vi "Th 1tache.vi"(3 "Indice tache":i8) -> (0 "données Th":string[](array[string]))   [LabVIEW 2022 SP3]
uses:
  <vilib>/DAQmx/read.llb/DAQmx Read (Analog 2D DBL NChan NSamp).vi
  <vilib>/Analysis/baseanly.llb/Mean (DBL).vi
  Variables globales/Variable glob Th.vi
  Variables globales/Variable glob generale.vi
  <vilib>/DAQmx/miscellaneous.llb/DAQmx Fill In Error Info.vi
  <resource>/objmgr/daqmx.rc
  <vilib>/Analysis/NI_AALBase.lvlib
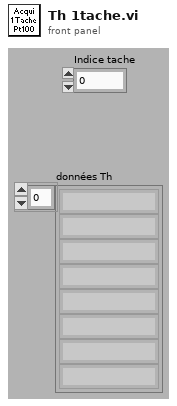
[diagram p1: front panel]
types:
  T1 = cluster{"Nom tache Th":refnum<k21>, "Noms des Th":string[], "Nb Th":i16, "Selection Th":bool[], "Nom Th selectionnes":string[]}[]
  T2 = cluster{"Nom tache Th":refnum<k21>, "Noms des Th":string[], "Nb Th":i16, "Selection Th":bool[], "Nom Th selectionnes":string[]}
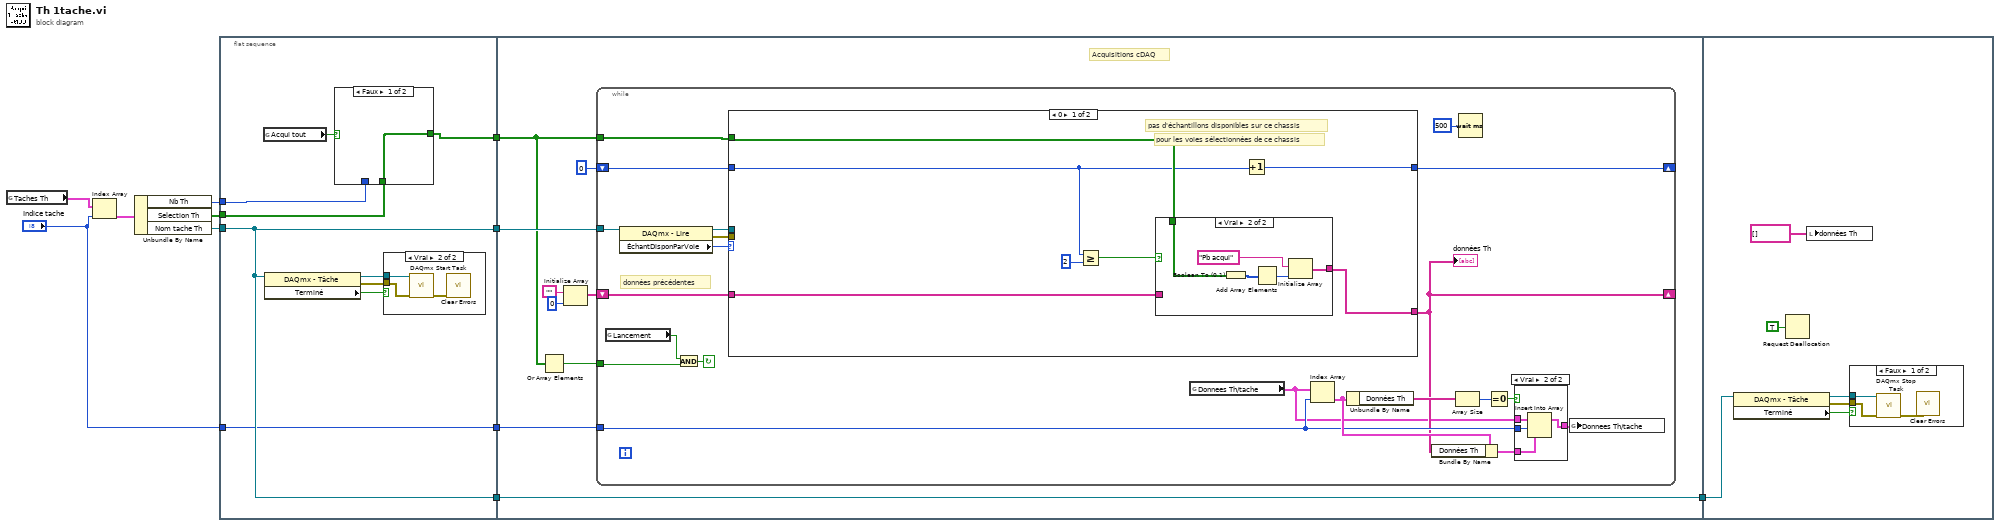
[diagram p0: block diagram]
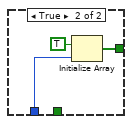
[diagram p3: hidden frame]
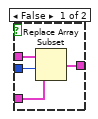
[diagram p4: hidden frame]
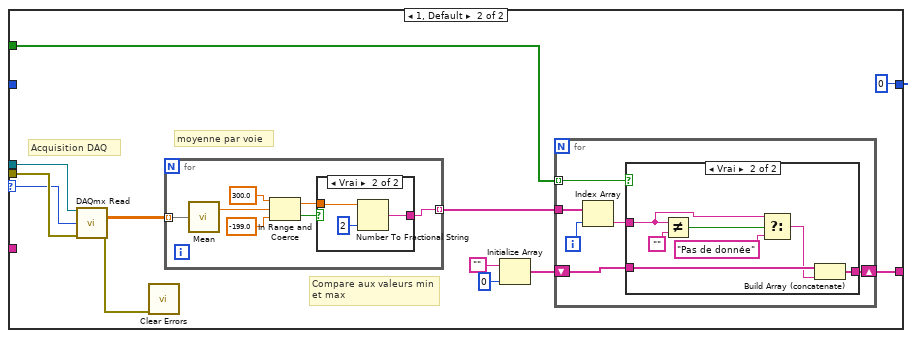
[diagram p6: hidden frame]
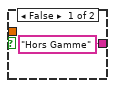
[diagram p8: hidden frame]
diagram:
  n1 = global read "Variable glob Th.vi" "Taches Th"() -> (w4:T1)
  n2 = Index Array(array=w4, index="Indice tache") -> (element=w3:T2)
  n3 = Unbundle By Name(w3) -> ("Nb Th"=w7:i16, "Selection Th"=w8:bool[], "Nom tache Th"=w9:refnum<k21>)
  n4 = flat-sequence {
    tunnel: [w19] -> w11
    tunnel: [w14] -> w10
    tunnel: w9 -> [w14]
    tunnel: w8 -> [w15]
    tunnel: w7 -> [w13]
    tunnel: [w14] -> w6
    tunnel: [w12] -> w2
    tunnel: "Indice tache" -> [w12]
    tunnel: w11 -> [w32]
    tunnel: w10 -> [w36]
    tunnel: w6 -> [w29]
    tunnel: [w29] -> w5
    tunnel: w2 -> [w28]
    tunnel: w5 -> [w117]
    frame #0 {
      n5 = global read "Variable glob generale.vi" "Acqui tout"() -> (w20:bool)
      n6 = property class="DAQmx - Tâche"(reference=w14) -> (reference out=w17:refnum<k21>, error out=w16:errorcluster, "Terminé"=w18:bool)  [unwired: 1 in]
      n7 = case shown="Faux" w20 {
        tunnel: [w24 w26] -> w19
        tunnel: w15 -> [w24 _]
        tunnel: w13 -> [_ w25]
        frame False {
        }
        frame True {
          n8 = Initialize Array(TRUE, w25) -> (w26:bool[])
        }
      }
      n9 = case shown="Vrai" w18 {
        tunnel: w17 -> [_ w23]
        tunnel: w16 -> [_ w22]
        frame False {
        }
        frame True {
          n10 = call <vilib>:"DAQmx Start Task.vi"("task/channels in"=w23, "error in"=w22) -> ("error out"=w21:errorcluster)  [unwired: 12 in, 1 out]
          n11 = call <vilib>:"Clear Errors.vi"("error in (no error)"=w21) -> ()  [unwired: 5 in, 2 out]
        }
      }
    }
    frame #1 {
      # "Acquisitions cDAQ"
      n12 = Or Array Elements(Boolean array=w32) -> (logical OR=w31:bool)
      n13 = Initialize Array("", 0 ("taille de la dimension")) -> (w33:string[])
      n14 = while {
        tunnel: w36 -> [w57]
        tunnel: w32 -> [w56]
        shift-right: [w38] -> _
        shift-left: w33 -> [w54]
        tunnel: w31 -> [w52]
        shift-right: [w47] -> _
        shift-left: 0 -> [w46]
        tunnel: w28 -> [w40]
        stop <- w51 continue-if-true
        # "données précédentes"
        n15 = global read "Variable glob generale.vi" "Lancement"() -> (w53:bool)
        n16 = property class="DAQmx - Lire"(reference=w57) -> (reference out=w50:refnum<k21>, error out=w48:errorcluster, "ÉchantDisponParVoie"=w49:u32)  [unwired: 1 in]
        n17 = And(x=w53, y=w52) -> (x .and. y?=w51:bool)
        n18 = case shown="0" w49 {
          selector: w49 -> [_ w79]
          tunnel: [w72 w80] -> w38
          tunnel: w56 -> [w71 w82]
          tunnel: w50 -> [_ w85]
          tunnel: w54 -> [w68 _]
          tunnel: w48 -> [_ w84]
          tunnel: [w70 0] -> w47
          tunnel: w46 -> [w69 _]
          frame 0 {
            # "pour les voies sélectionnées de ce chassis"
            # "pas d'échantillons disponibles sur ce chassis"
            n19 = Greater Or Equal?(x=w69, y=2) -> (x >= y?=w66:bool)
            n20 = case shown="Vrai" w66 {
              tunnel: [w73 w74] -> w72
              tunnel: w71 -> [_ w77]
              tunnel: w68 -> [w73 _]
              frame False {
              }
              frame True {
                n21 = Boolean To (0,1)(Boolean=w77) -> (0, 1=w76:i16[])
                n22 = Add Array Elements(numeric array=w76) -> (sum=w75:i16)
                n23 = Initialize Array("Pb acqui", w75) -> (w74:string[])
              }
            }
            n24 = Increment(x=w69) -> (x+1=w70:i32)
          }
          frame 1, Default {
            # "Acquisition DAQ"
            # "moyenne par voie"
            # "Compare aux valeurs min et max"
            n25 = call-poly <vilib>:"DAQmx Read.vi"("task/channels in"=w85, "number of samples per channel"=w79, "error in"=w84) -> ("data"=w89:dbl[][], "error out"=w83:errorcluster)  [unwired: 10 in, 1 out]
            n26 = call <vilib>:"Clear Errors.vi"("error in (no error)"=w83) -> ()  [unwired: 5 in, 2 out]
            n27 = for {
              tunnel: w89 -> [w111] mode=indexing
              tunnel: [w105] -> w90 mode=indexing
              n28 = call-poly <vilib>:"Mean.vi"("X"=w111) -> ("mean"=w108:dbl)  [unwired: 1 out]
              n29 = In Range and Coerce(upper limit=300.0 ("élément"), x=w108, lower limit=-199.0 ("élément")) -> (coerced(x)=w106:dbl, In Range?=w107:bool)
              n30 = case shown="Vrai" w107 {
                tunnel: w106 -> [_ w114]
                tunnel: ["Hors Gamme" w113] -> w105
                frame False {
                }
                frame True {
                  n31 = Number To Fractional String(number=w114, precision (6)=i16 2 ("précision (6)")) -> (F-format string=w113:string)  [unwired: 2 in]
                }
              }
            }
            n32 = Initialize Array("", 0 ("taille de la dimension")) -> (w88:string[])
            n33 = for {
              tunnel: w82 -> [w96] mode=indexing
              tunnel: w90 -> [w95]
              shift-right: [w91] -> w80
              shift-left: w88 -> [w92]
              i -> [w94]
              n34 = Index Array(array=w95, index=w94) -> (element=w93:string)
              n35 = case shown="Vrai" w96 {
                tunnel: w93 -> [_ w103]
                tunnel: w92 -> [w97 w101]
                tunnel: [w97 w100] -> w91
                frame False {
                  # "voie non sélectionnée"
                }
                frame True {
                  n36 = Not Equal?(x=w103, y="") -> (x != y?=w98:bool)
                  n37 = Select(t=w103, s=w98, f="Pas de donnée" ("cas faux")) -> (s? t:f=w99:string)
                  n38 = Build Array (concatenate)(w101, w99) -> (w100:string[])
                }
              }
            }
          }
        }
        "données Th" <- w38
        n39 = global read "Variable glob Th.vi" "Donnees Th/tache"() -> (w37:cluster{"Données Th":string[]}[])
        n40 = Index Array(array=w37, index=w40) -> (element=w42:cluster{"Données Th":string[]})
        n41 = Unbundle By Name(w42) -> ("Données Th"=w39:string[])
        n42 = Bundle By Name(cluster=w42, "Données Th"=w38) -> (w41:cluster{"Données Th":string[]})
        n43 = Array Size(array=w39) -> (size(s)=w45:i32)
        n44 = Wait (ms)(milliseconds to wait=u32 500 ("n millisecondes")) -> ()  [unwired: 1 out]
        n45 = Equal To 0?(x=w45) -> (x = 0?=w44:bool)
        n46 = case shown="Vrai" w44 {
          tunnel: w41 -> [w61 w65]
          tunnel: [w60 w62] -> w43
          tunnel: w37 -> [w59 w64]
          tunnel: w40 -> [w58 w63]
          frame False {
            n47 = Replace Array Subset(array=w59, new element=w61, index=w58) -> (w60:cluster{"Données Th":string[]}[])
          }
          frame True {
            n48 = Insert Into Array(array=w64, index=w63, new element=w65) -> (w62:cluster{"Données Th":string[]}[])
          }
        }
        n49 = global write "Variable glob Th.vi" "Donnees Th/tache"(w43) -> ()
      }
    }
    frame #2 {
      n50 = property class="DAQmx - Tâche"(reference=w117) -> (reference out=w119:refnum<k21>, error out=w118:errorcluster, "Terminé"=w120:bool)  [unwired: 1 in]
      n51 = Request Deallocation(TRUE ("flag")) -> ()
      n52 = local write "données Th"(string[] [] ("Données Pt 1D")) -> ()
      n53 = case shown="Faux" w120 {
        tunnel: w119 -> [w124 _]
        tunnel: w118 -> [w123 _]
        frame False {
          n54 = call <vilib>:"DAQmx Stop Task.vi"("task/channels in"=w124, "error in"=w123) -> ("error out"=w122:errorcluster)  [unwired: 12 in, 1 out]
          n55 = call <vilib>:"Clear Errors.vi"("error in (no error)"=w122) -> ()  [unwired: 5 in, 2 out]
        }
        frame True {
        }
      }
    }
  }
